vi "plcm3ChannelSetting.vi"(0 "Handle In":i16, 1 "CH1 Measurement Type":u32(ring)=1 items=["OFF", "1mV range (1mV/A)", "10mV range (10mV/A)", "100mV range (100mV/A)", "Voltage Input"], 2 "CH2 Measurement Type":u32(ring) items=["OFF", "1mV range (1mV/A)", "10mV range (10mV/A)", "100mV range (100mV/A)", "Voltage Input"], 3 "CH3 Measurement Type":u32(ring) items=["OFF", "1mV range (1mV/A)", "10mV range (10mV/A)", "100mV range (100mV/A)", "Voltage Input"], 11 "error in (no error)":errorcluster) -> (4 "Handle out":i16, 6 "Channel Enable Array":u8[](array[numeric]), 15 "error out":errorcluster)   [LabVIEW 2010]
uses:
  plcm3.dll
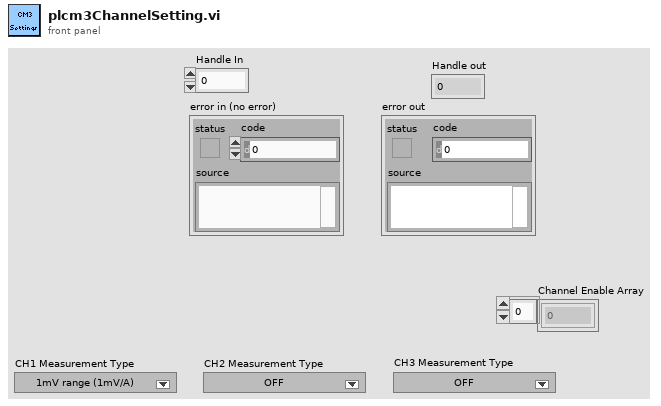
[diagram p1: front panel]
types:
  T1 = cluster{"status":bool, "code":u32, "source":string}
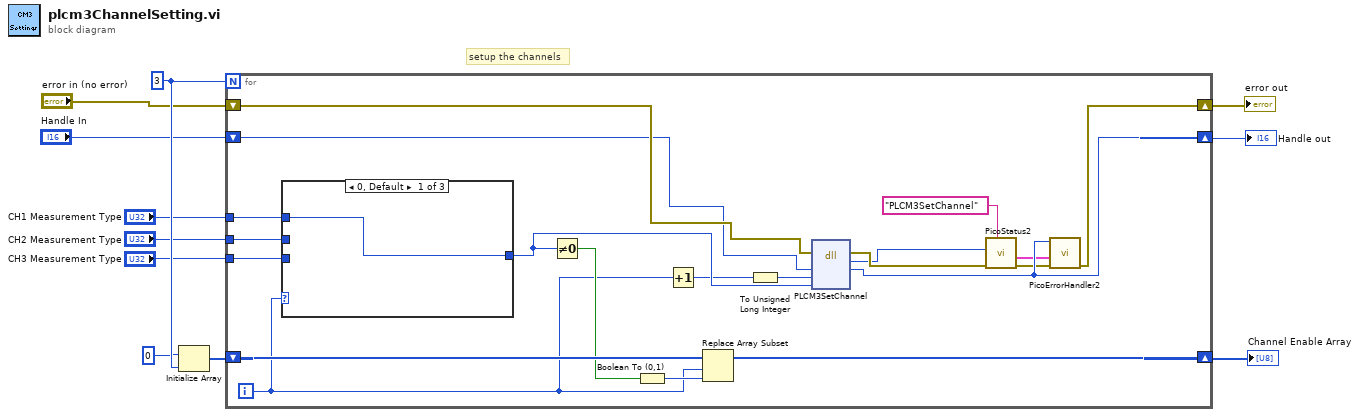
[diagram p0: block diagram]
diagram:
  w10 = 3
  # "setup the channels"
  n1 = Initialize Array(u8 0 ("element"), w10) -> (w8:u8[])
  n2 = for {
    N: w10 -> [_]
    shift-right: [w31] -> w11
    shift-left: w8 -> [w30]
    shift-right: [w26] -> w7
    shift-left: "Handle In" -> [w24]
    shift-right: [w27] -> w4
    shift-left: "error in (no error)" -> [w25]
    tunnel: "CH1 Measurement Type" -> [w23]
    tunnel: "CH2 Measurement Type" -> [w21]
    tunnel: "CH3 Measurement Type" -> [w20]
    i -> [w17]
    n3 = case shown="0, Default" w17 {
      tunnel: [w32 w33 w34] -> w22
      tunnel: w23 -> [w32 _ _]
      tunnel: w21 -> [_ w33 _]
      tunnel: w20 -> [_ _ w34]
      frame 0, Default {
      }
      frame 1 {
      }
      frame 2 {
      }
    }
    n4 = Not Equal To 0?(x=w22) -> (x != 0?=w28:bool)
    n5 = Boolean To (0,1)(Boolean=w28) -> (0, 1=w29:i16)
    n6 = Increment(x=w17) -> (x+1=w18:i32)
    n7 = Replace Array Subset(array=w30, new element=w29, index=w17) -> (w31:u8[])
    n8 = To Unsigned Long Integer(number=w18) -> (unsigned 32bit integer=w19:u32)
    n9 = dll-call lib="PLCM3.dll" fn="PLCM3SetChannel"(error in=w25, "handle"=w24, "channel"=w19, "type"=w22) -> (error out=w13:errorcluster, "PICO_STATUS"=w12:u32, "handle"=w26:i16)  [unwired: 4 in, 1 out]
    n10 = call "PicoStatus2.vi"("PICO source"="PLCM3SetChannel" ("source"), "Error in"=w13, "PICO STATUS"=w12) -> ("error out"=w16:errorcluster, "PICO_STATUS out"=w15:T1)  [unwired: 5 in]
    n11 = call "PicoErrorHandler2.vi"("error in (no error)"=w16, "PICO_STATUS in"=w15, "handle In"=w26) -> ("error out"=w27:errorcluster)  [unwired: 8 in]
  }
  "Channel Enable Array" <- w11
  "Handle out" <- w7
  "error out" <- w4
